vi "Labview_trieur_balles.vi"(8 "error in (no error)":errorcluster, 10 "Numeric":i32) -> (0 "error out":errorcluster)   [LabVIEW 2017]
uses:
  enum_trieur_balle.ctl
  <vilib>/Platform/TimedLoop/XDataNode/XDataNode.xnode
  <vilib>/Platform/TimedLoop/XDataNode/nitl_modes.ctl
  <vilib>/Platform/TimedLoop/XDataNode/XDNodeRunTimeDep.lvlib
  <vilib>/Platform/TimedLoop/XDataNode/wakeup.ctl
  <vilib>/Platform/TimedLoop/XDataNode/timing_clust.ctl
panel:
  in  "delay rotation 6":i32=38000
  in  "delay rotation 5":i32=37000
  in  "delay rotation 4":i32=36000
  in  "delay rotation 3":i32=36500
  in  "delay rotation 2":i32=36000
  in  "delay rotation":i32=39000
  in  "x 2":i32=10000000
  in  "x":i32=10000000
  out "x+1 4":i32
  out "Couleur 4":bool
  out "Cluster 4":T1
  out "x+1 3":i32
  out "Couleur 3":bool
  out "Cluster 3":T1
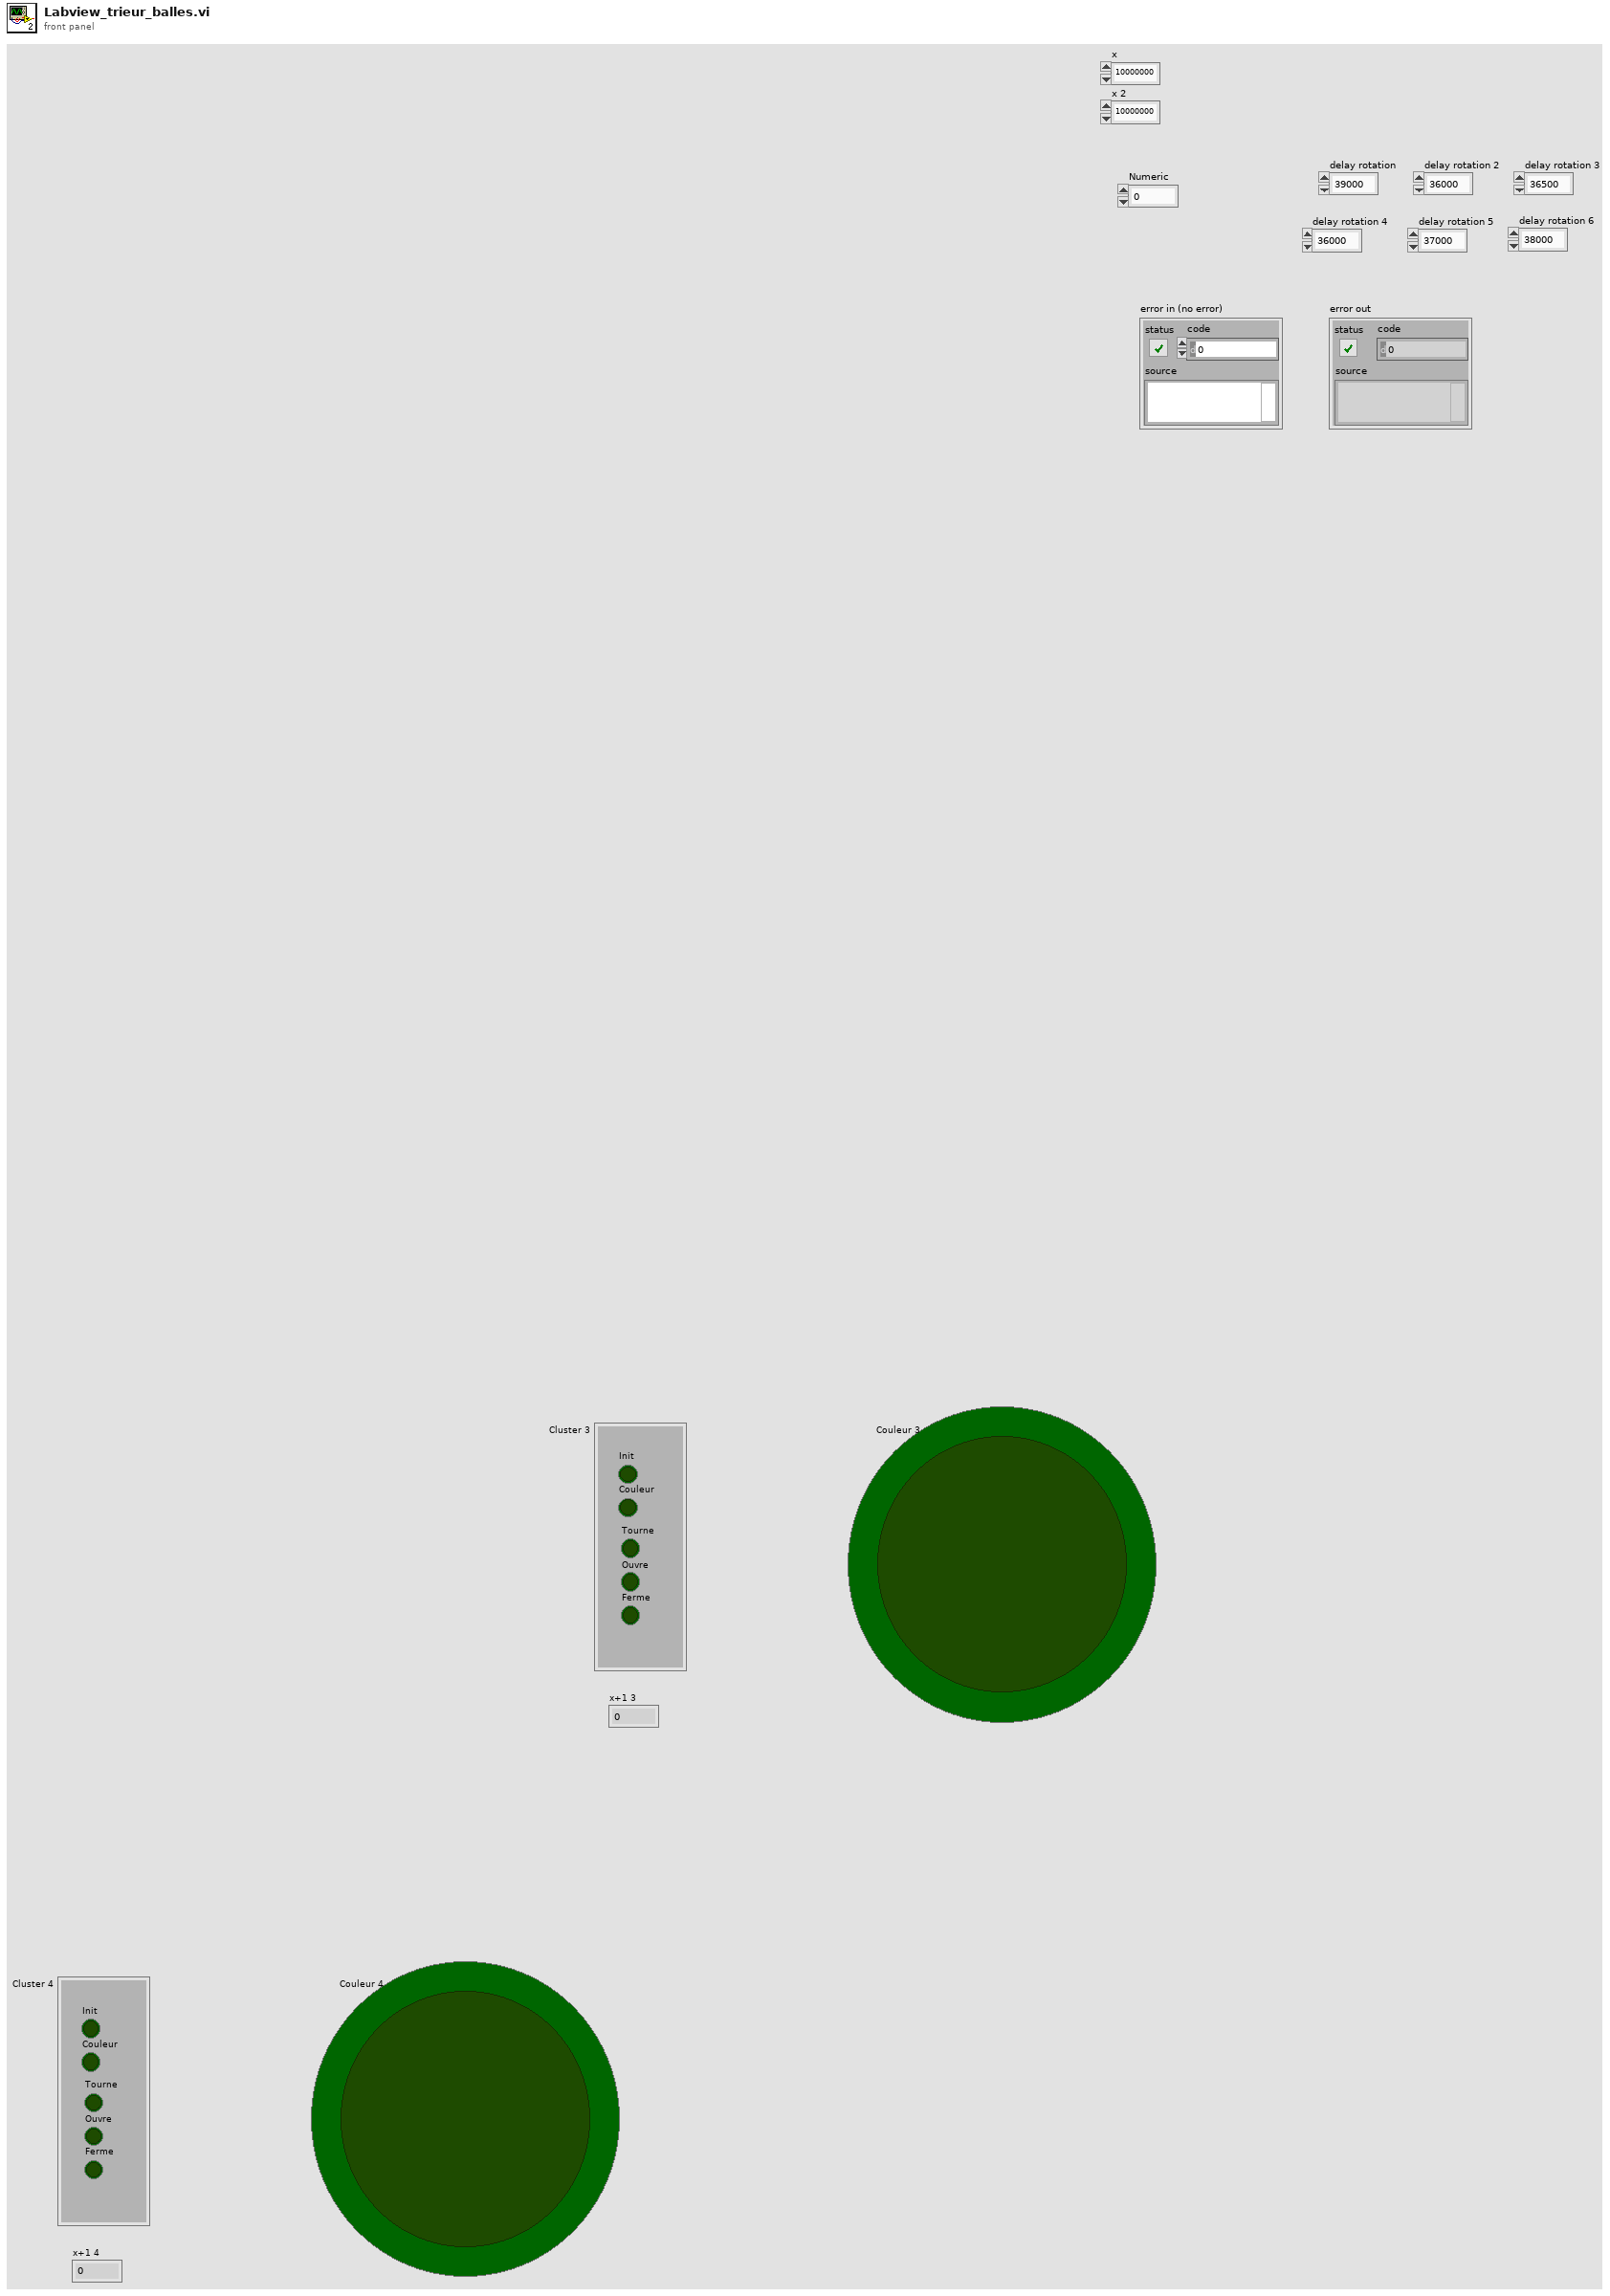
[diagram p1: front panel]
types:
  T1 = cluster{"Init":bool, "Couleur":bool, "Tourne":bool, "Ouvre":bool, "Ferme":bool}
  T2 = typedef "enum_trieur_balle.ctl" = enum16{"Initialisation", "Couleur", "Rotation", "Ouverture", "Fermeture"}
  T3 = cluster{"Booléen":bool, "Booléen 2":bool, "Booléen 3":bool, "Booléen 4":bool, "Booléen 5":bool}
  T4 = typedef "XDNodeRunTimeDep.lvlib/timing_clust.ctl" = cluster{"Expected End [f-1]":u64, "Actual End [f-1]":u64, "Finished Late? [f-1]":bool, "Expected End [i-1]":u64, "Actual End [i-1]":u64, "Finished Late? [i-1]":bool, "Expected Start [i]":u64, "Actual Start [i]":u64, "Expected Start [f]":u64, "Actual Start [f]":u64, "Source Name":string, "Structure Name":string, "Period":i64, "Deadline":i64, "Offset":i64, "Start":i64, "Priority":i32, "Timeout":i32, "Mode":T5, "Wakeup Reason":T6, "Error":errorcluster, "Source Type":string, "Secondary Source Type":string, "Global End Time":u64, "Global Start Time":u64, "Frame Duration":u64, "Iteration Duration":u64, "Assigned CPU":i32, "I/O Scan Engine Mode":u32}
  T5 = typedef "XDNodeRunTimeDep.lvlib/nitl_modes.ctl" = enum32{"No Change", "Process missed periods, maintain original phase", "Discard missed periods, maintain original phase", "Process missed periods, ignore original phase", "Discard missed periods, ignore original phase"}
  T6 = typedef "XDNodeRunTimeDep.lvlib/wakeup.ctl" = enum32{"Normal", "Aborted", "Asynchronous wakeup", "Timing source error", "Timed loop error", "Timeout"}
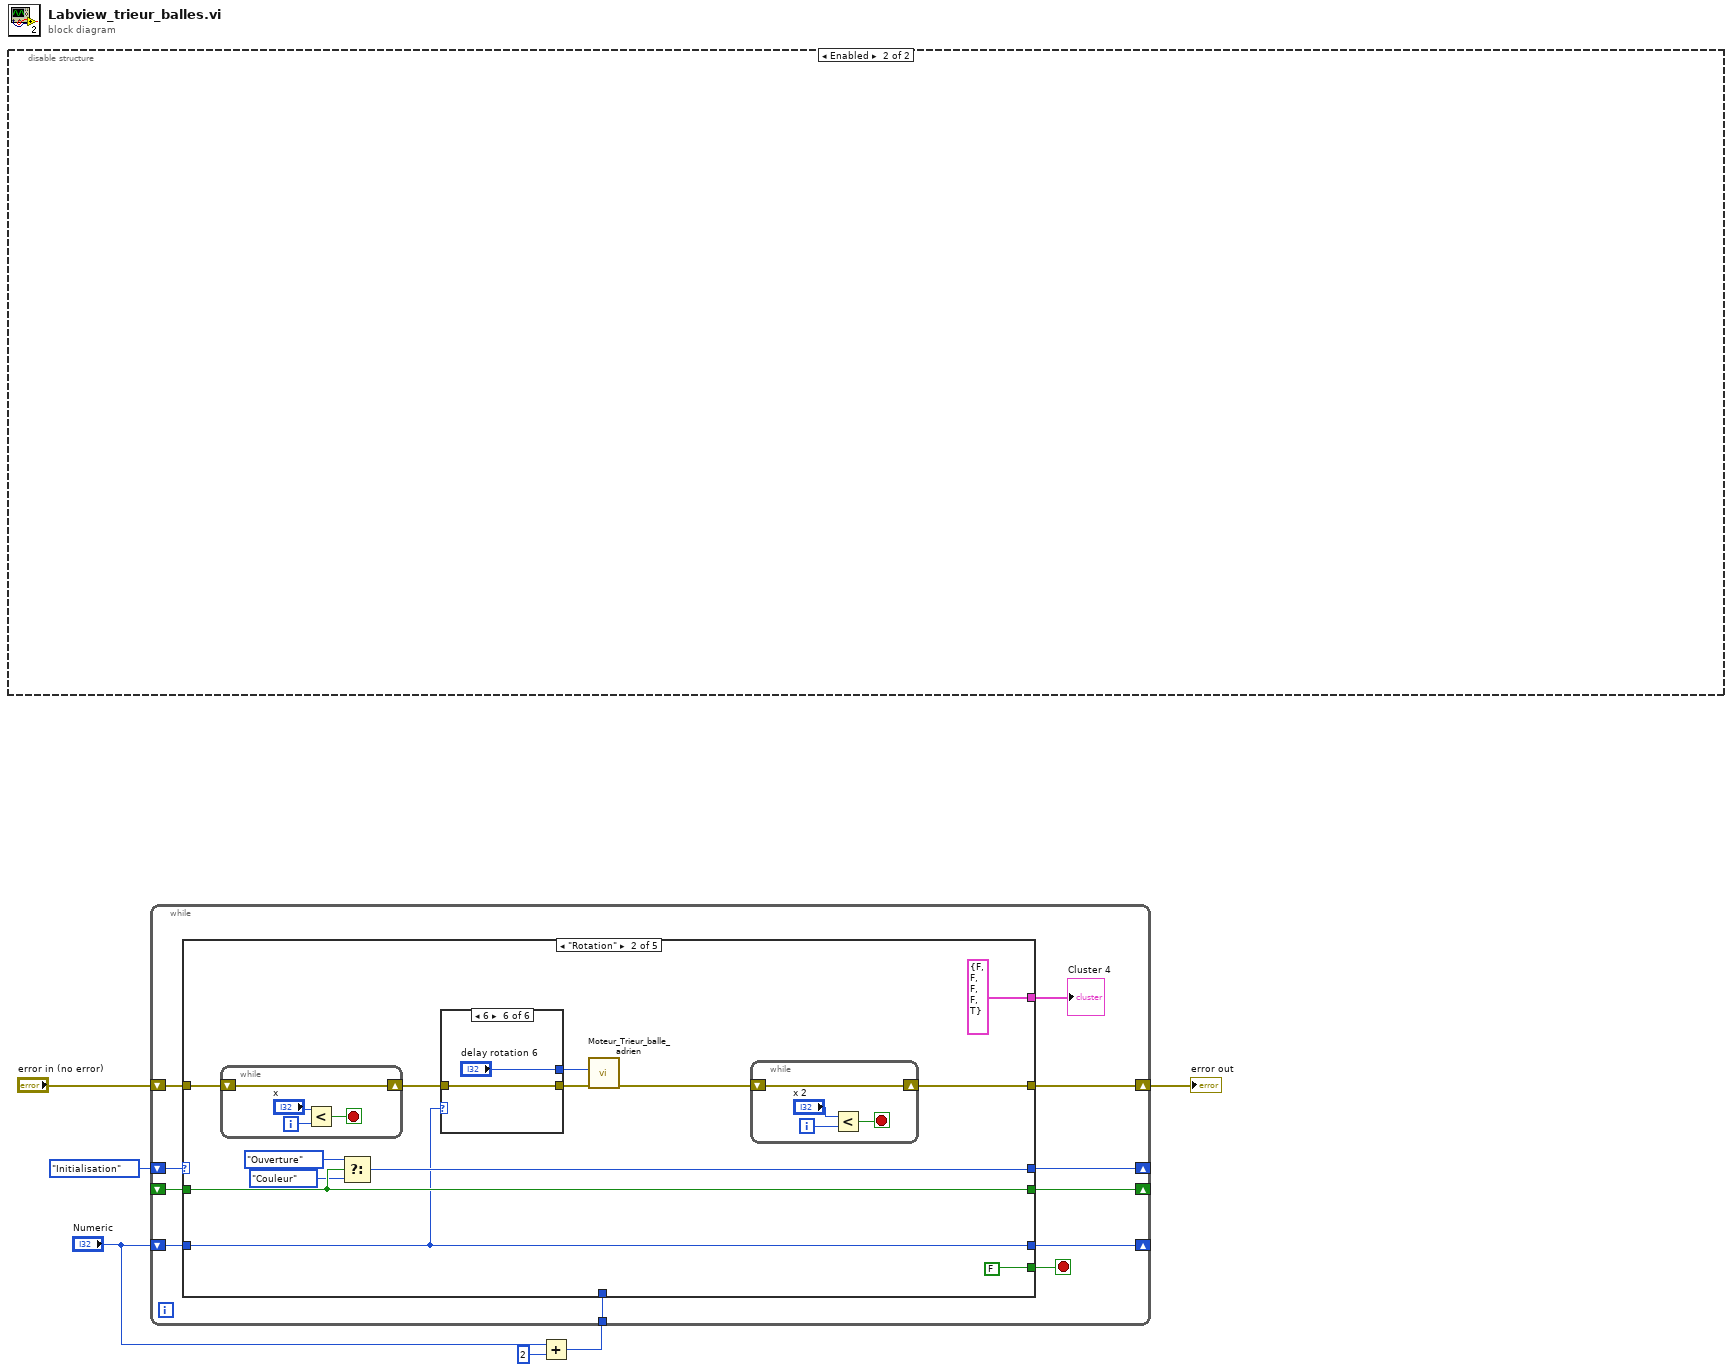
[diagram p0: block diagram]
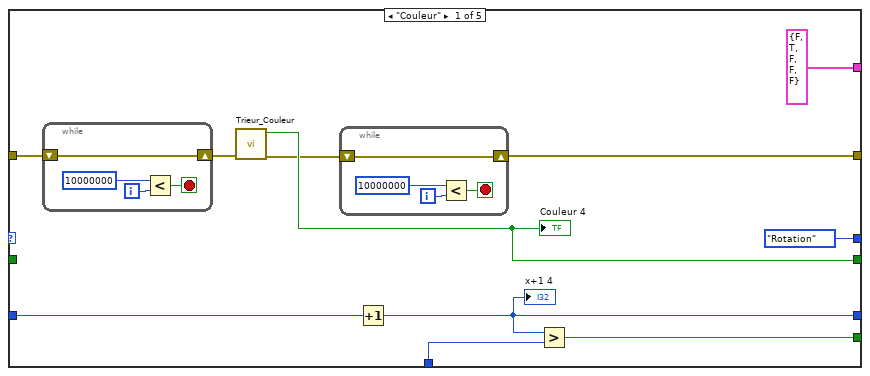
[diagram p2: hidden frame]
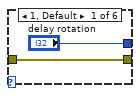
[diagram p3: hidden frame]
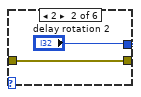
[diagram p4: hidden frame]
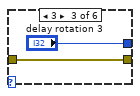
[diagram p5: hidden frame]
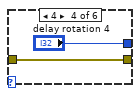
[diagram p6: hidden frame]
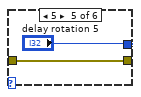
[diagram p7: hidden frame]
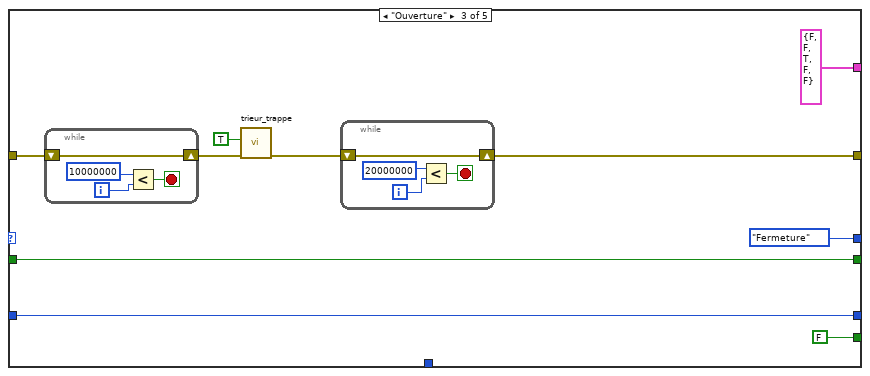
[diagram p8: hidden frame]
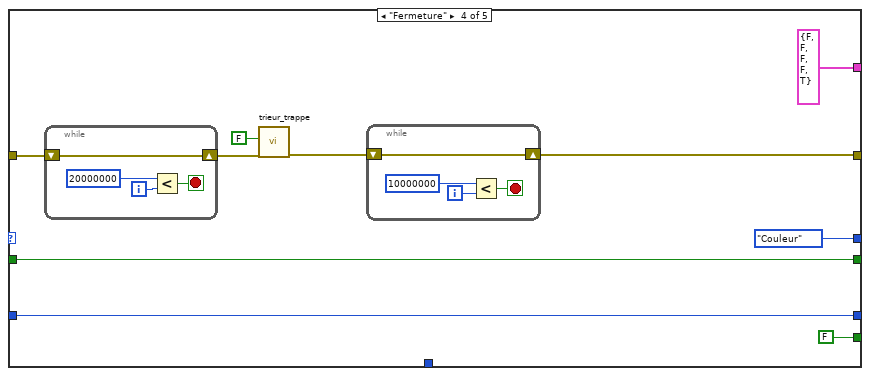
[diagram p9: hidden frame]
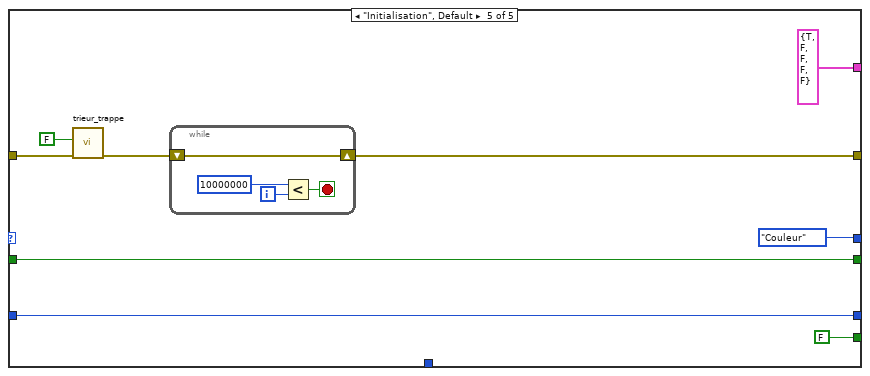
[diagram p10: hidden frame]
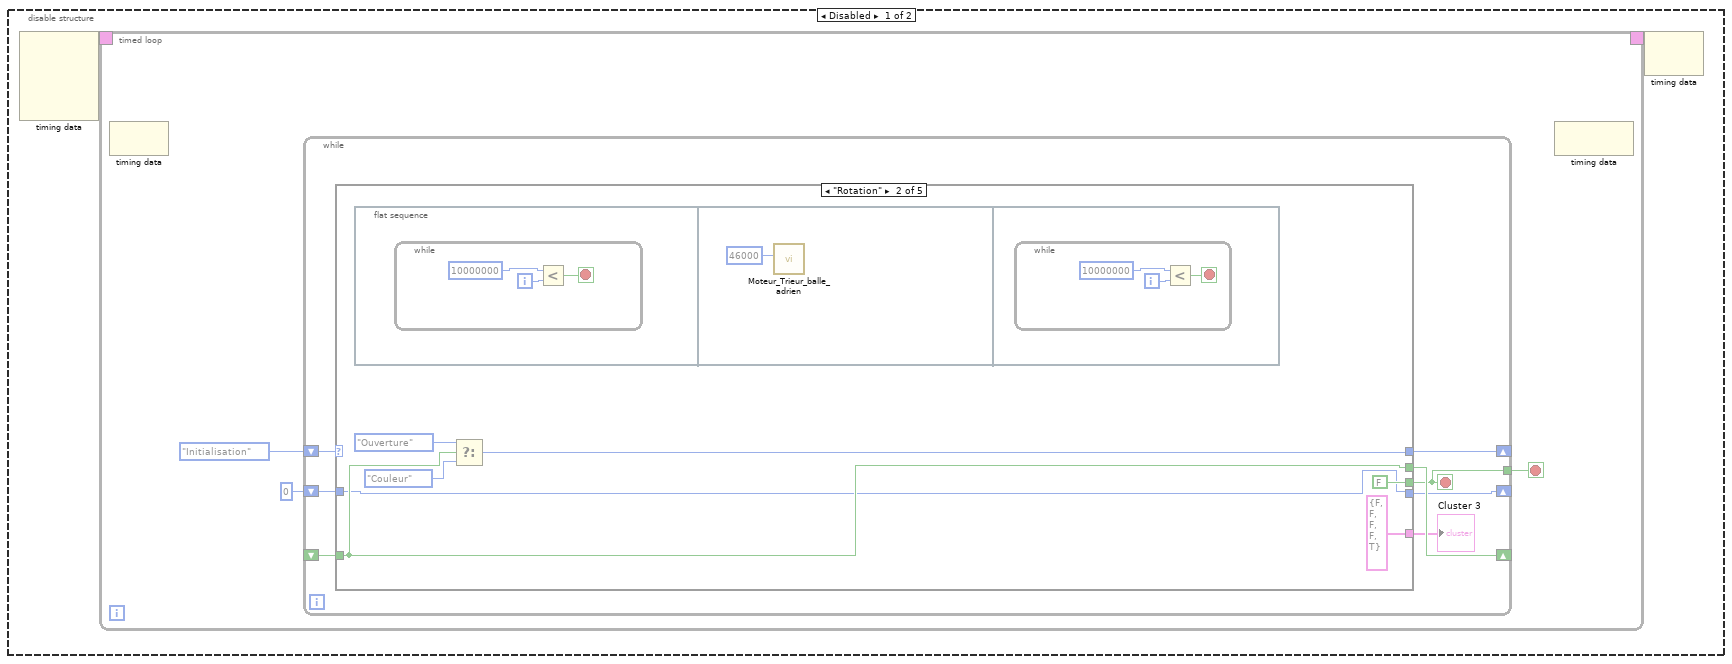
[diagram p11: hidden frame]
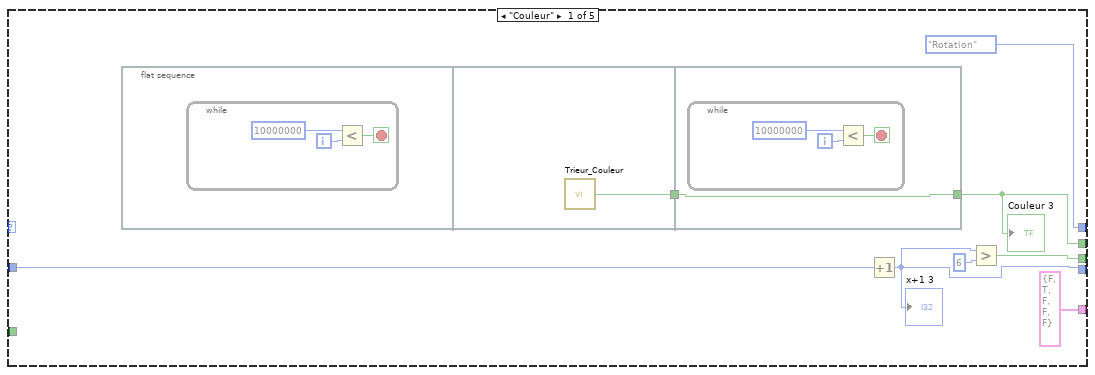
[diagram p12: hidden frame]
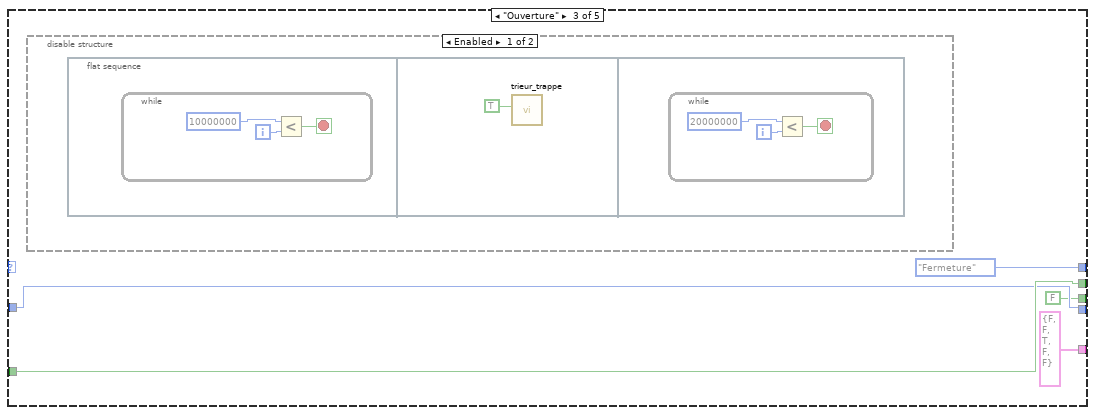
[diagram p13: hidden frame]
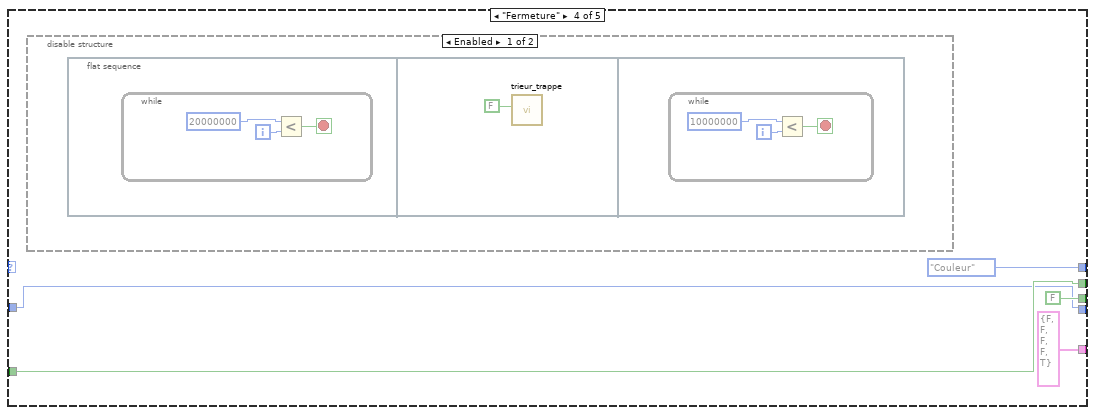
[diagram p15: hidden frame]
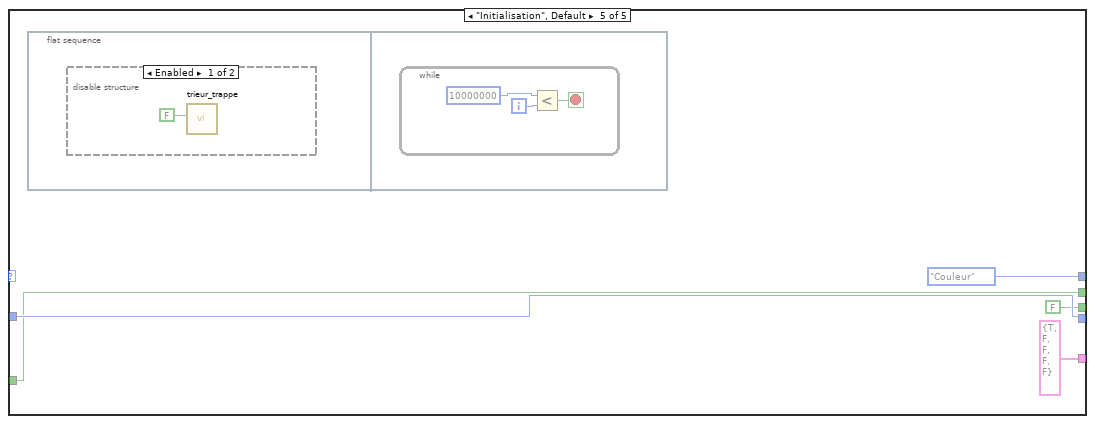
[diagram p17: hidden frame]
diagram:
  n1 = disable-structure shown="Enabled" {
    frame Disabled {
      n2 = node-c288() -> (w8:T4)  [unwired: 4 in]
      n3 = timed-loop {
        timing: w8 -> [_]
        timing-out: [_] -> w7
        stop <- w9 stop-if-true
        n4 = node-c288() -> ()  [unwired: 1 in, 1 out]
        n5 = while {
          shift-right: [w15] -> _
          shift-left: enum_trieur_balle."Initialisation" -> [w19]
          shift-right: [w18] -> _
          shift-left: _ -> [w14]
          shift-right: [w16] -> _
          shift-left: 0 -> [w17]
          tunnel: [w12] -> w9
          stop <- w12 stop-if-true
          n6 = case shown="\"Rotation\"" w19 {
            tunnel: [w21 w40 w54 w65 w75] -> w18
            tunnel: w17 -> [w27 w39 w53 w64 w78]
            tunnel: [w24 w39 w53 w64 w78] -> w16
            tunnel: [w22 FALSE FALSE FALSE FALSE] -> w12
            tunnel: [enum_trieur_balle."Rotation" w41 enum_trieur_balle."Fermeture" enum_trieur_balle."Couleur" enum_trieur_balle."Couleur"] -> w15
            tunnel: w14 -> [_ w40 w54 w65 w75]
            tunnel: [T3 {"Booléen"=FALSE, "Booléen 2"=TRUE, "Booléen 3"=FALSE, "Booléen 4"=FALSE, "Booléen 5"=FALSE} ("Cluster") T3 {"Booléen"=FALSE, "Booléen 2"=FALSE, "Booléen 3"=FALSE, "Booléen 4"=FALSE, "Booléen 5"=TRUE} ("Cluster") T3 {"Booléen"=FALSE, "Booléen 2"=FALSE, "Booléen 3"=TRUE, "Booléen 4"=FALSE, "Booléen 5"=FALSE} ("Cluster") T3 {"Booléen"=FALSE, "Booléen 2"=FALSE, "Booléen 3"=FALSE, "Booléen 4"=FALSE, "Booléen 5"=TRUE} ("Cluster") T3 {"Booléen"=TRUE, "Booléen 2"=FALSE, "Booléen 3"=FALSE, "Booléen 4"=FALSE, "Booléen 5"=FALSE} ("Cluster")] -> w13
            frame "Couleur" {
              n7 = flat-sequence {
                tunnel: [w31] -> w20
                tunnel: [w32] -> w21
                tunnel: w20 -> [w32]
                frame #0 {
                  n8 = while {
                    i -> [w30]
                    stop <- w28 stop-if-true
                    n9 = Less?(x=10000000, y=w30) -> (x < y?=w28:bool)
                  }
                }
                frame #1 {
                  n10 = call "Trieur_Couleur.vi"() -> ("Couleur"=w31:bool)  [unwired: 2 in]
                }
                frame #2 {
                  n11 = while {
                    i -> [w35]
                    stop <- w33 stop-if-true
                    n12 = Less?(x=10000000, y=w35) -> (x < y?=w33:bool)
                  }
                }
              }
              n13 = Increment(x=w27) -> (x+1=w24:i32)
              "x+1 3" <- w24
              n14 = Greater?(x=w24, y=6) -> (0:w22:bool)
              "Couleur 3" <- w21
            }
            frame "Rotation" {
              n15 = flat-sequence {
                frame #0 {
                  n16 = while {
                    i -> [w45]
                    stop <- w43 stop-if-true
                    n17 = Less?(x=10000000, y=w45) -> (x < y?=w43:bool)
                  }
                }
                frame #1 {
                  n18 = call "Moteur_Trieur_balle_adrien.vi"("delay rotation"=46000) -> ()  [unwired: 10 in, 1 out]
                }
                frame #2 {
                  n19 = while {
                    i -> [w49]
                    stop <- w47 stop-if-true
                    n20 = Less?(x=10000000, y=w49) -> (x < y?=w47:bool)
                  }
                }
              }
              n21 = Select(t=enum_trieur_balle."Ouverture", s=w40, f=enum_trieur_balle."Couleur") -> (s? t:f=w41:T2)
            }
            frame "Ouverture" {
              n22 = disable-structure shown="Enabled" {
                frame Enabled {
                  n23 = flat-sequence {
                    frame #0 {
                      n24 = while {
                        i -> [w57]
                        stop <- w55 stop-if-true
                        n25 = Less?(x=10000000, y=w57) -> (x < y?=w55:bool)
                      }
                    }
                    frame #1 {
                      n26 = call "trieur_trappe.vi"("Ouvrir"=TRUE) -> ()  [unwired: 10 in, 1 out]
                    }
                    frame #2 {
                      n27 = while {
                        i -> [w61]
                        stop <- w59 stop-if-true
                        n28 = Less?(x=20000000, y=w61) -> (x < y?=w59:bool)
                      }
                    }
                  }
                }
                frame Disabled {
                }
              }
            }
            frame "Fermeture" {
              n29 = disable-structure shown="Enabled" {
                frame Enabled {
                  n30 = flat-sequence {
                    frame #0 {
                      n31 = while {
                        i -> [w69]
                        stop <- w67 stop-if-true
                        n32 = Less?(x=20000000, y=w69) -> (x < y?=w67:bool)
                      }
                    }
                    frame #1 {
                      n33 = call "trieur_trappe.vi"("Ouvrir"=FALSE) -> ()  [unwired: 10 in, 1 out]
                    }
                    frame #2 {
                      n34 = while {
                        i -> [w73]
                        stop <- w71 stop-if-true
                        n35 = Less?(x=10000000, y=w73) -> (x < y?=w71:bool)
                      }
                    }
                  }
                }
                frame Disabled {
                }
              }
            }
            frame "Initialisation", Default {
              n36 = flat-sequence {
                frame #0 {
                  n37 = disable-structure shown="Enabled" {
                    frame Enabled {
                      n38 = call "trieur_trappe.vi"("Ouvrir"=FALSE) -> ()  [unwired: 10 in, 1 out]
                    }
                    frame Disabled {
                    }
                  }
                }
                frame #1 {
                  n39 = while {
                    i -> [w82]
                    stop <- w80 stop-if-true
                    n40 = Less?(x=10000000, y=w82) -> (x < y?=w80:bool)
                  }
                }
              }
            }
          }
          "Cluster 3" <- w13
        }
        n41 = node-c288() -> ()  [unwired: 1 in, 1 out]
      }
      n42 = node-c288(w7) -> ()  [unwired: 1 out]
    }
    frame Enabled {
    }
  }
  n43 = Add(x="Numeric", y=2) -> (x+y=w3:i32)
  n44 = while {
    shift-right: [w93] -> _
    shift-left: enum_trieur_balle."Initialisation" -> [w97]
    shift-right: [w96] -> _
    shift-left: _ -> [w92]
    shift-right: [w94] -> _
    shift-left: "Numeric" -> [w95]
    tunnel: w3 -> [w89]
    shift-right: [w87] -> w1
    shift-left: "error in (no error)" -> [w88]
    stop <- w90 stop-if-true
    n45 = case shown="\"Rotation\"" w97 {
      tunnel: [w103 w127 w159 w176 w191] -> w96
      tunnel: w95 -> [w108 w123 w158 w175 w194]
      tunnel: [w105 w123 w158 w175 w194] -> w94
      tunnel: [w104 FALSE FALSE FALSE FALSE] -> w90
      tunnel: [enum_trieur_balle."Rotation" w128 enum_trieur_balle."Fermeture" enum_trieur_balle."Couleur" enum_trieur_balle."Couleur"] -> w93
      tunnel: w92 -> [_ w127 w159 w176 w191]
      tunnel: [T3 {"Booléen"=FALSE, "Booléen 2"=TRUE, "Booléen 3"=FALSE, "Booléen 4"=FALSE, "Booléen 5"=FALSE} ("Cluster") T3 {"Booléen"=FALSE, "Booléen 2"=FALSE, "Booléen 3"=FALSE, "Booléen 4"=FALSE, "Booléen 5"=TRUE} ("Cluster") T3 {"Booléen"=FALSE, "Booléen 2"=FALSE, "Booléen 3"=TRUE, "Booléen 4"=FALSE, "Booléen 5"=FALSE} ("Cluster") T3 {"Booléen"=FALSE, "Booléen 2"=FALSE, "Booléen 3"=FALSE, "Booléen 4"=FALSE, "Booléen 5"=TRUE} ("Cluster") T3 {"Booléen"=TRUE, "Booléen 2"=FALSE, "Booléen 3"=FALSE, "Booléen 4"=FALSE, "Booléen 5"=FALSE} ("Cluster")] -> w91
      tunnel: w89 -> [w102 _ _ _ _]
      tunnel: w88 -> [w101 w121 w153 w171 w188]
      tunnel: [w98 w117 w150 w168 w186] -> w87
      frame "Couleur" {
        n46 = while {
          shift-right: [w113] -> w100
          shift-left: w101 -> [w113]
          i -> [w116]
          stop <- w114 stop-if-true
          n47 = Less?(x=10000000, y=w116) -> (x < y?=w114:bool)
        }
        n48 = call "Trieur_Couleur.vi"("error in (no error)"=w100) -> ("error out"=w99:errorcluster, "Couleur"=w103:bool)  [unwired: 7 in]
        "Couleur 4" <- w103
        n49 = while {
          shift-right: [w109] -> w98
          shift-left: w99 -> [w109]
          i -> [w112]
          stop <- w110 stop-if-true
          n50 = Less?(x=10000000, y=w112) -> (x < y?=w110:bool)
        }
        n51 = Increment(x=w108) -> (x+1=w105:i32)
        "x+1 4" <- w105
        n52 = Greater?(x=w105, y=w102) -> (0:w104:bool)
      }
      frame "Rotation" {
        n53 = while {
          shift-right: [w146] -> w119
          shift-left: w121 -> [w146]
          i -> [w149]
          stop <- w148 stop-if-true
          n54 = Less?(x="x", y=w149) -> (x < y?=w148:bool)
        }
        n55 = Select(t=enum_trieur_balle."Ouverture", s=w127, f=enum_trieur_balle."Couleur") -> (s? t:f=w128:T2)
        n56 = case shown="6" w123 {
          tunnel: ["delay rotation" "delay rotation 2" "delay rotation 3" "delay rotation 4" "delay rotation 5" "delay rotation 6"] -> w122
          tunnel: [w134 w136 w138 w140 w142 w144] -> w120
          tunnel: w119 -> [w134 w136 w138 w140 w142 w144]
          frame 1, Default {
          }
          frame 2 {
          }
          frame 3 {
          }
          frame 4 {
          }
          frame 5 {
          }
          frame 6 {
          }
        }
        n57 = call "Moteur_Trieur_balle_adrien.vi"("error in (no error)"=w120, "delay rotation"=w122) -> ("error out"=w118:errorcluster)  [unwired: 9 in]
        n58 = while {
          shift-right: [w130] -> w117
          shift-left: w118 -> [w130]
          i -> [w133]
          stop <- w132 stop-if-true
          n59 = Less?(x="x 2", y=w133) -> (x < y?=w132:bool)
        }
      }
      frame "Ouverture" {
        n60 = while {
          shift-right: [w164] -> w152
          shift-left: w153 -> [w164]
          i -> [w167]
          stop <- w165 stop-if-true
          n61 = Less?(x=10000000, y=w167) -> (x < y?=w165:bool)
        }
        n62 = call "trieur_trappe.vi"("error in (no error)"=w152, "Ouvrir"=TRUE) -> ("error out"=w151:errorcluster)  [unwired: 9 in]
        n63 = while {
          shift-right: [w160] -> w150
          shift-left: w151 -> [w160]
          i -> [w163]
          stop <- w161 stop-if-true
          n64 = Less?(x=20000000, y=w163) -> (x < y?=w161:bool)
        }
      }
      frame "Fermeture" {
        n65 = while {
          shift-right: [w182] -> w170
          shift-left: w171 -> [w182]
          i -> [w185]
          stop <- w183 stop-if-true
          n66 = Less?(x=20000000, y=w185) -> (x < y?=w183:bool)
        }
        n67 = call "trieur_trappe.vi"("error in (no error)"=w170, "Ouvrir"=FALSE) -> ("error out"=w169:errorcluster)  [unwired: 9 in]
        n68 = while {
          shift-right: [w178] -> w168
          shift-left: w169 -> [w178]
          i -> [w181]
          stop <- w179 stop-if-true
          n69 = Less?(x=10000000, y=w181) -> (x < y?=w179:bool)
        }
      }
      frame "Initialisation", Default {
        n70 = call "trieur_trappe.vi"("error in (no error)"=w188, "Ouvrir"=FALSE) -> ("error out"=w187:errorcluster)  [unwired: 9 in]
        n71 = while {
          shift-right: [w195] -> w186
          shift-left: w187 -> [w195]
          i -> [w198]
          stop <- w196 stop-if-true
          n72 = Less?(x=10000000, y=w198) -> (x < y?=w196:bool)
        }
      }
    }
    "Cluster 4" <- w91
  }
  "error out" <- w1
